vi "Read library name.vi"(8 "error in":errorcluster, 11 "editorscriptingobject in":refnum<class "editorscriptingobjectadv.lvclass">) -> (0 "error out":errorcluster, 2 "library name":string, 3 "editorscriptingobject out":refnum<class "editorscriptingobjectadv.lvclass">)   [LabVIEW 2014, in "editorscriptingobjectadv.lvclass"]
uses:
  editorscriptingobjectadv.lvclass
  editorscriptingobjectadv.lvclass/editorscriptingobjectadv.ctl
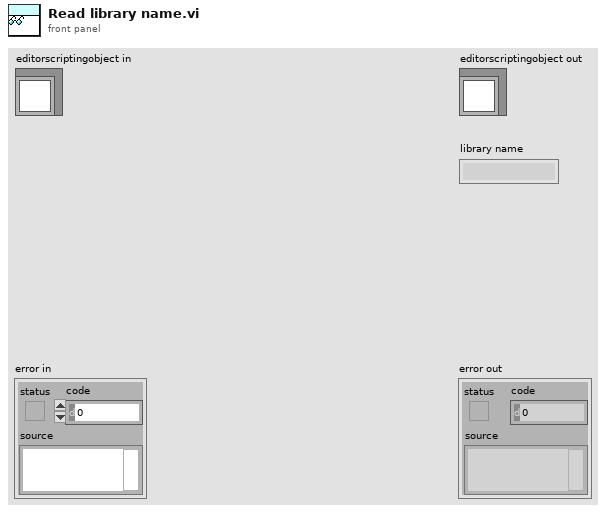
[diagram p1: front panel]
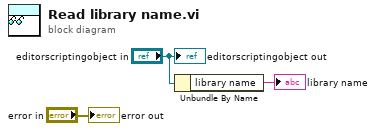
[diagram p0: block diagram]
diagram:
  n1 = Unbundle By Name("editorscriptingobject in") -> ("library name"=→"library name":string)
  "error out" <- "error in"
  "editorscriptingobject out" <- "editorscriptingobject in"
